vi "clust.vi"(11 "VISA resource name":refnum<visa-resource-name>) -> (2 "Cluster":T1 {"Slide" scale=0.0..100.0})   [LabVIEW 2017]
uses:
  Control 2.ctl
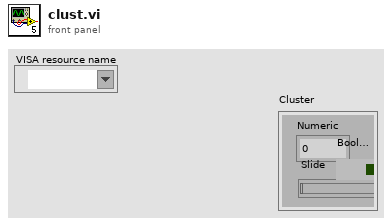
[diagram p1: front panel]
types:
  T1 = typedef "Control 2.ctl" = cluster{"Numeric":dbl, "Slide":u8, "Boolean":bool}
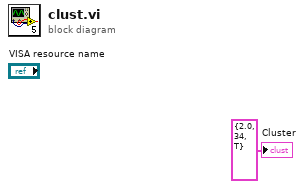
[diagram p0: block diagram]
diagram:
  "Cluster" <- T1 {"Numeric"=2.0, "Slide"=34, "Boolean"=TRUE} ("Cluster")
